vi "Test Plant First Order Step A.vi"(8 "error in":errorcluster) -> (0 "error out":errorcluster)   [LabVIEW 2026]
doc: "Caraya test of Plant First Order Step.vi: one step per channel and all channels (FOS-1..4). Expected values from TEST_CASES.md, abs tol 1e-6."
uses:
  <vilib>/addons/_JKI Toolkits/Caraya/classes/Test/Test.lvclass
  <vilib>/addons/_JKI Toolkits/Caraya/classes/Assert/Assert.lvclass
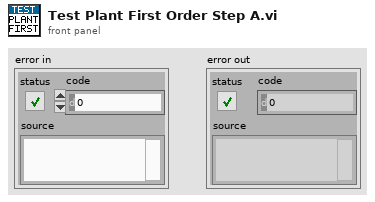
[diagram p1: front panel]
types:
  T1 = cluster{"pressure_sp_bar":dbl, "flow_sp_lpm":dbl, "displacement_sp_mm":dbl}
  T2 = cluster{"pressure_bar":dbl, "flow_lpm":dbl, "displacement_mm":dbl, "timestamp_ms":dbl}
  T3 = typedef "Plant Feedback.ctl" = cluster{"pressure_bar":dbl, "flow_lpm":dbl, "displacement_mm":dbl, "timestamp_ms":dbl}
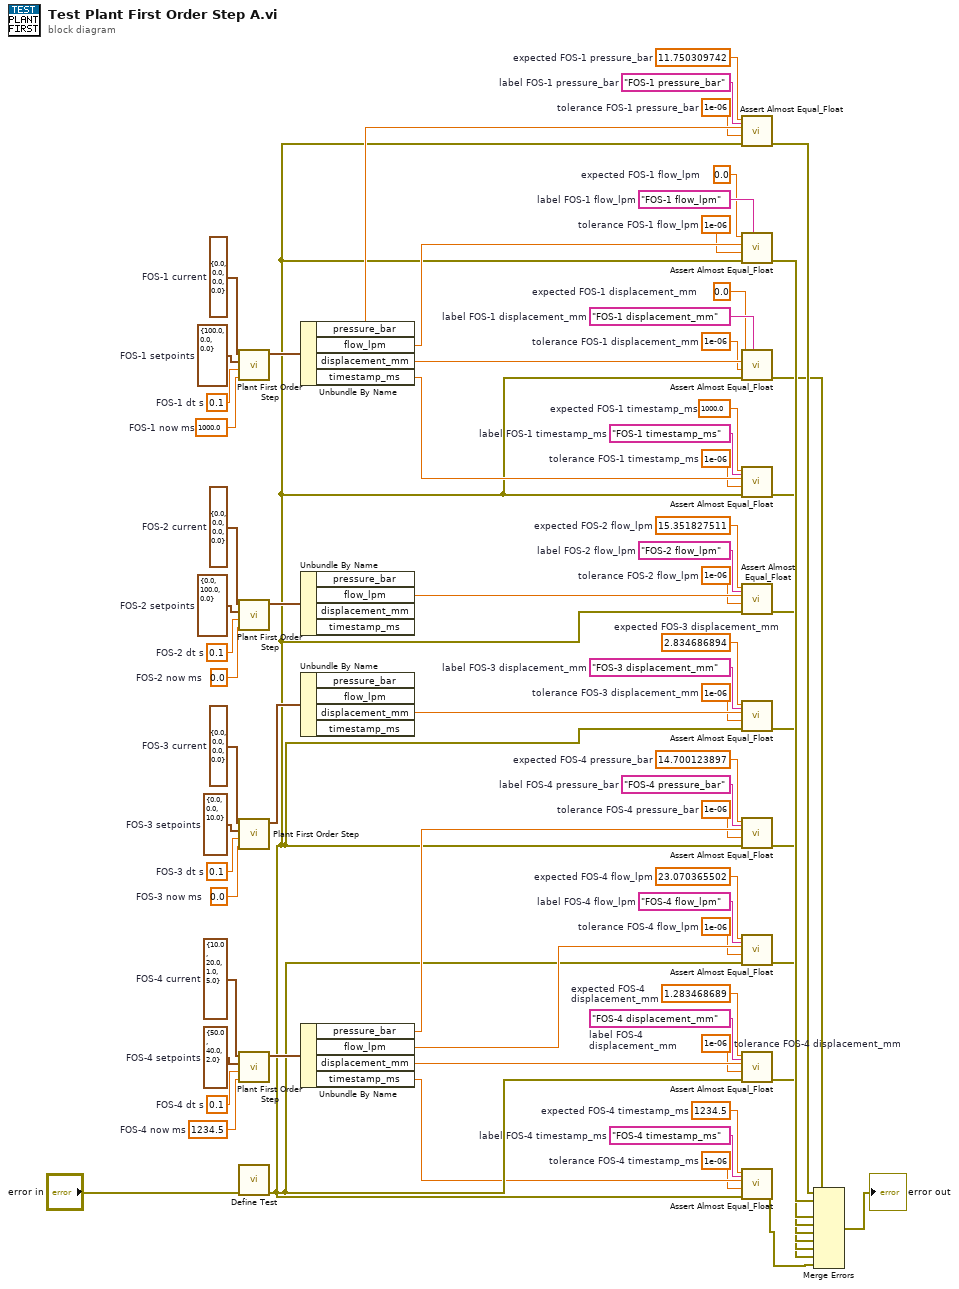
[diagram p0: block diagram]
diagram:
  w16 = "FOS-4 timestamp_ms"  # label FOS-4 timestamp_ms
  w12 = 1e-06  # tolerance FOS-4 timestamp_ms
  w14 = 1234.5  # expected FOS-4 timestamp_ms
  w20 = "FOS-4 displacement_mm"  # label FOS-4 displacement_mm
  w17 = 1e-06  # tolerance FOS-4 displacement_mm
  w19 = 1.283468689  # expected FOS-4 displacement_mm
  w24 = "FOS-4 flow_lpm"  # label FOS-4 flow_lpm
  w21 = 1e-06  # tolerance FOS-4 flow_lpm
  w23 = 23.070365502  # expected FOS-4 flow_lpm
  w28 = "FOS-4 pressure_bar"  # label FOS-4 pressure_bar
  w25 = 1e-06  # tolerance FOS-4 pressure_bar
  w27 = 14.700123897  # expected FOS-4 pressure_bar
  w30 = 1234.5  # FOS-4 now ms
  w31 = 0.1  # FOS-4 dt s
  w32 = T1 {"pressure_sp_bar"=50.0, "flow_sp_lpm"=40.0, "displacement_sp_mm"=2.0}  # FOS-4 setpoints
  w33 = T2 {"pressure_bar"=10.0, "flow_lpm"=20.0, "displacement_mm"=1.0, "timestamp_ms"=5.0}  # FOS-4 current
  w37 = "FOS-3 displacement_mm"  # label FOS-3 displacement_mm
  w34 = 1e-06  # tolerance FOS-3 displacement_mm
  w36 = 2.834686894  # expected FOS-3 displacement_mm
  w39 = 0.0  # FOS-3 now ms
  w40 = 0.1  # FOS-3 dt s
  w41 = T1 {"pressure_sp_bar"=0.0, "flow_sp_lpm"=0.0, "displacement_sp_mm"=10.0}  # FOS-3 setpoints
  w42 = T2 {"pressure_bar"=0.0, "flow_lpm"=0.0, "displacement_mm"=0.0, "timestamp_ms"=0.0}  # FOS-3 current
  w46 = "FOS-2 flow_lpm"  # label FOS-2 flow_lpm
  w43 = 1e-06  # tolerance FOS-2 flow_lpm
  w45 = 15.351827511  # expected FOS-2 flow_lpm
  w48 = 0.0  # FOS-2 now ms
  w49 = 0.1  # FOS-2 dt s
  w50 = T1 {"pressure_sp_bar"=0.0, "flow_sp_lpm"=100.0, "displacement_sp_mm"=0.0}  # FOS-2 setpoints
  w51 = T2 {"pressure_bar"=0.0, "flow_lpm"=0.0, "displacement_mm"=0.0, "timestamp_ms"=0.0}  # FOS-2 current
  w55 = "FOS-1 timestamp_ms"  # label FOS-1 timestamp_ms
  w52 = 1e-06  # tolerance FOS-1 timestamp_ms
  w54 = 1000.0  # expected FOS-1 timestamp_ms
  w59 = "FOS-1 displacement_mm"  # label FOS-1 displacement_mm
  w56 = 1e-06  # tolerance FOS-1 displacement_mm
  w58 = 0.0  # expected FOS-1 displacement_mm
  w63 = "FOS-1 flow_lpm"  # label FOS-1 flow_lpm
  w60 = 1e-06  # tolerance FOS-1 flow_lpm
  w62 = 0.0  # expected FOS-1 flow_lpm
  w67 = "FOS-1 pressure_bar"  # label FOS-1 pressure_bar
  w64 = 1e-06  # tolerance FOS-1 pressure_bar
  w66 = 11.750309742  # expected FOS-1 pressure_bar
  w69 = 1000.0  # FOS-1 now ms
  w70 = 0.1  # FOS-1 dt s
  w71 = T1 {"pressure_sp_bar"=100.0, "flow_sp_lpm"=0.0, "displacement_sp_mm"=0.0}  # FOS-1 setpoints
  w72 = T2 {"pressure_bar"=0.0, "flow_lpm"=0.0, "displacement_mm"=0.0, "timestamp_ms"=0.0}  # FOS-1 current
  n1 = call "Plant First Order Step.vi"("now ms"=w69, "dt s"=w70, "Plant Setpoints"=w71, "current Plant Feedback"=w72) -> ("new Plant Feedback"=w68:T3)  [unwired: 7 in]
  n2 = call "Plant First Order Step.vi"("now ms"=w48, "dt s"=w49, "Plant Setpoints"=w50, "current Plant Feedback"=w51) -> ("new Plant Feedback"=w47:T3)  [unwired: 7 in]
  n3 = call "Plant First Order Step.vi"("now ms"=w39, "dt s"=w40, "Plant Setpoints"=w41, "current Plant Feedback"=w42) -> ("new Plant Feedback"=w38:T3)  [unwired: 7 in]
  n4 = call "Plant First Order Step.vi"("now ms"=w30, "dt s"=w31, "Plant Setpoints"=w32, "current Plant Feedback"=w33) -> ("new Plant Feedback"=w29:T3)  [unwired: 7 in]
  n5 = call <vilib>:"Define Test.vi"("error in (no error)"="error in") -> ("error out"=w15:errorcluster)  [unwired: 9 in, 1 out]
  n6 = Unbundle By Name(w68) -> ("pressure_bar"=w65:dbl, "flow_lpm"=w61:dbl, "displacement_mm"=w57:dbl, "timestamp_ms"=w53:dbl)
  n7 = Unbundle By Name(w47) -> ("flow_lpm"=w44:dbl)  [unwired: 3 out]
  n8 = Unbundle By Name(w38) -> ("displacement_mm"=w35:dbl)  [unwired: 3 out]
  n9 = Unbundle By Name(w29) -> ("pressure_bar"=w26:dbl, "flow_lpm"=w22:dbl, "displacement_mm"=w18:dbl, "timestamp_ms"=w13:dbl)
  n10 = call <vilib>:"Assert Almost Equal_Float.vi"("Label"=w67, "error in (no error)"=w15, "Tolerance"=w64, "Actual"=w65, "Expected"=w66) -> ("error out"=w11:errorcluster)  [unwired: 5 in, 1 out]
  n11 = call <vilib>:"Assert Almost Equal_Float.vi"("Label"=w63, "error in (no error)"=w15, "Tolerance"=w60, "Actual"=w61, "Expected"=w62) -> ("error out"=w10:errorcluster)  [unwired: 5 in, 1 out]
  n12 = call <vilib>:"Assert Almost Equal_Float.vi"("Label"=w59, "error in (no error)"=w15, "Tolerance"=w56, "Actual"=w57, "Expected"=w58) -> ("error out"=w9:errorcluster)  [unwired: 5 in, 1 out]
  n13 = call <vilib>:"Assert Almost Equal_Float.vi"("Label"=w55, "error in (no error)"=w15, "Tolerance"=w52, "Actual"=w53, "Expected"=w54) -> ("error out"=w8:errorcluster)  [unwired: 5 in, 1 out]
  n14 = call <vilib>:"Assert Almost Equal_Float.vi"("Label"=w46, "error in (no error)"=w15, "Tolerance"=w43, "Actual"=w44, "Expected"=w45) -> ("error out"=w7:errorcluster)  [unwired: 5 in, 1 out]
  n15 = call <vilib>:"Assert Almost Equal_Float.vi"("Label"=w37, "error in (no error)"=w15, "Tolerance"=w34, "Actual"=w35, "Expected"=w36) -> ("error out"=w6:errorcluster)  [unwired: 5 in, 1 out]
  n16 = call <vilib>:"Assert Almost Equal_Float.vi"("Label"=w28, "error in (no error)"=w15, "Tolerance"=w25, "Actual"=w26, "Expected"=w27) -> ("error out"=w5:errorcluster)  [unwired: 5 in, 1 out]
  n17 = call <vilib>:"Assert Almost Equal_Float.vi"("Label"=w24, "error in (no error)"=w15, "Tolerance"=w21, "Actual"=w22, "Expected"=w23) -> ("error out"=w4:errorcluster)  [unwired: 5 in, 1 out]
  n18 = call <vilib>:"Assert Almost Equal_Float.vi"("Label"=w20, "error in (no error)"=w15, "Tolerance"=w17, "Actual"=w18, "Expected"=w19) -> ("error out"=w3:errorcluster)  [unwired: 5 in, 1 out]
  n19 = call <vilib>:"Assert Almost Equal_Float.vi"("Label"=w16, "error in (no error)"=w15, "Tolerance"=w12, "Actual"=w13, "Expected"=w14) -> ("error out"=w2:errorcluster)  [unwired: 5 in, 1 out]
  n20 = Merge Errors(w11, w10, w9, w8, w7, w6, w5, w4, w3, w2) -> (→"error out":errorcluster)
